vi "PicoScope6000Settings.vi"(4 "Channel D Settings":T2 {"Bandwidth" items=["Full", "20 MHz"]; "Range" items=["10 mV", "20 mV", "50 mV", "100 mV", "200 mV", "500 mV", "1 V", "2 V", "5 V", "10 V", "20 V", "50 V ", "100 V"]; "Coupling" items=["AC", "DC 1 MOhm", "DC 50 Ohm"]}, 5 "Channel B Settings":T2 {"Bandwidth" items=["Full", "20 MHz"]; "Range" items=["10 mV", "20 mV", "50 mV", "100 mV", "200 mV", "500 mV", "1 V", "2 V", "5 V", "10 V", "20 V", "50 V ", "100 V"]; "Coupling" items=["AC", "DC 1 MOhm", "DC 50 Ohm"]}, 6 "Channel C Settings":T2 {"Bandwidth" items=["Full", "20 MHz"]; "Range" items=["10 mV", "20 mV", "50 mV", "100 mV", "200 mV", "500 mV", "1 V", "2 V", "5 V", "10 V", "20 V", "50 V ", "100 V"]; "Coupling" items=["AC", "DC 1 MOhm", "DC 50 Ohm"]}, 7 "Channel A Settings":T2 {"Bandwidth" items=["Full", "20 MHz"]; "Range" items=["10 mV", "20 mV", "50 mV", "100 mV", "200 mV", "500 mV", "1 V", "2 V", "5 V", "10 V", "20 V", "50 V ", "100 V"]; "Coupling" items=["AC", "DC 1 MOhm", "DC 50 Ohm"]}, 8 "error in":errorcluster, 9 "Device Info":T1, 10 "Trigger Settings":T3 {"Trigger Direction" items=["Rising", "Falling"]}, 11 "handle in":i16) -> (0 "error out":errorcluster, 1 "Enabled array":i16[](array[numeric]), 3 "handle out":i16)   [LabVIEW 2009]
doc: "This VI is used to set up the oscilloscope. The inputs are clusters for setting channel and simple trigger settings. Advanced triggers can be set up using PicoScope6000AdvancedTriggerSettings.vi"
uses:
  ps6000.dll
  PicoScope6000AnalogChannelSettings.ctl
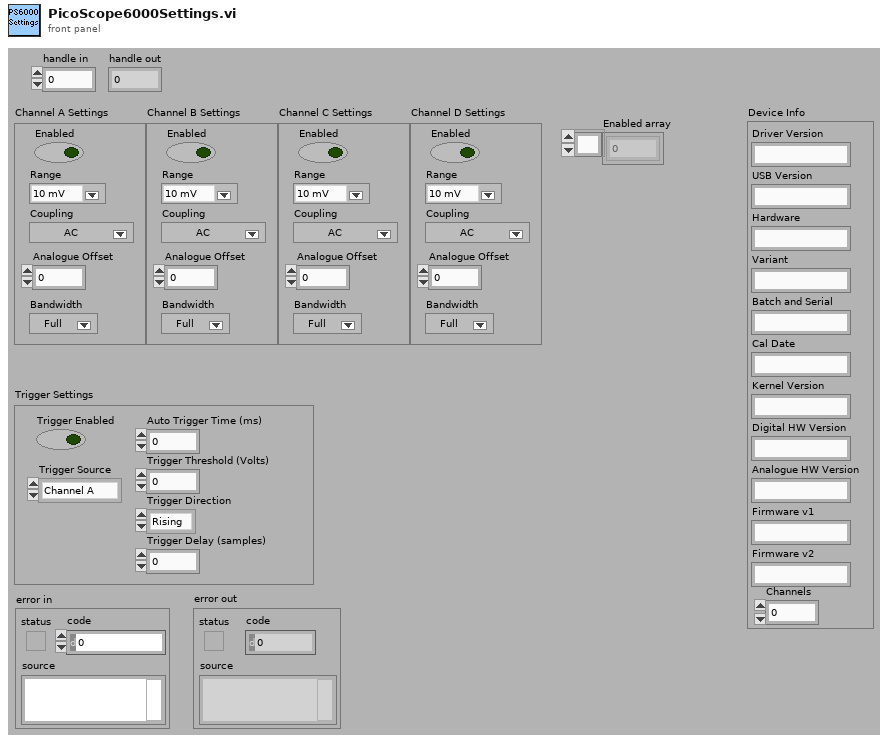
[diagram p1: front panel]
types:
  T1 = cluster{"Driver Version":string, "USB Version":string, "Hardware":string, "Variant":string, "Batch and Serial":string, "Cal Date":string, "Kernel Version":string, "Digital HW Version":string, "Analogue HW Version":string, "Firmware v1":string, "Firmware v2":string, "Channels":i16}
  T2 = typedef "PicoScope6000AnalogChannelSettings.ctl" = cluster{"Enabled":bool, "Coupling":u32, "Range":u32, "Analogue Offset":sgl, "Bandwidth":u32}
  T3 = cluster{"Trigger Enabled":bool, "Trigger Source":enum32{"Channel A", "Channel B", "Channel C", "Channel D", "External", "Aux."}, "Trigger Threshold (Volts)":dbl, "Trigger Direction":u16, "Trigger Delay (samples)":u32, "Auto Trigger Time (ms)":i16}
  T4 = cluster{"Enabled":bool, "Coupling":i32, "Range":u16, "Analogue Offset":sgl, "Bandwidth":i32}
  T5 = cluster{"Enabled":bool, "Coupling":u32, "Range":u32, "Analogue Offset":sgl, "Bandwidth":u32}
  T6 = cluster{"status":bool, "code":u32, "source":string}
  T7 = enum32{"Channel A", "Channel B", "Channel C", "Channel D", "External", "Aux."}
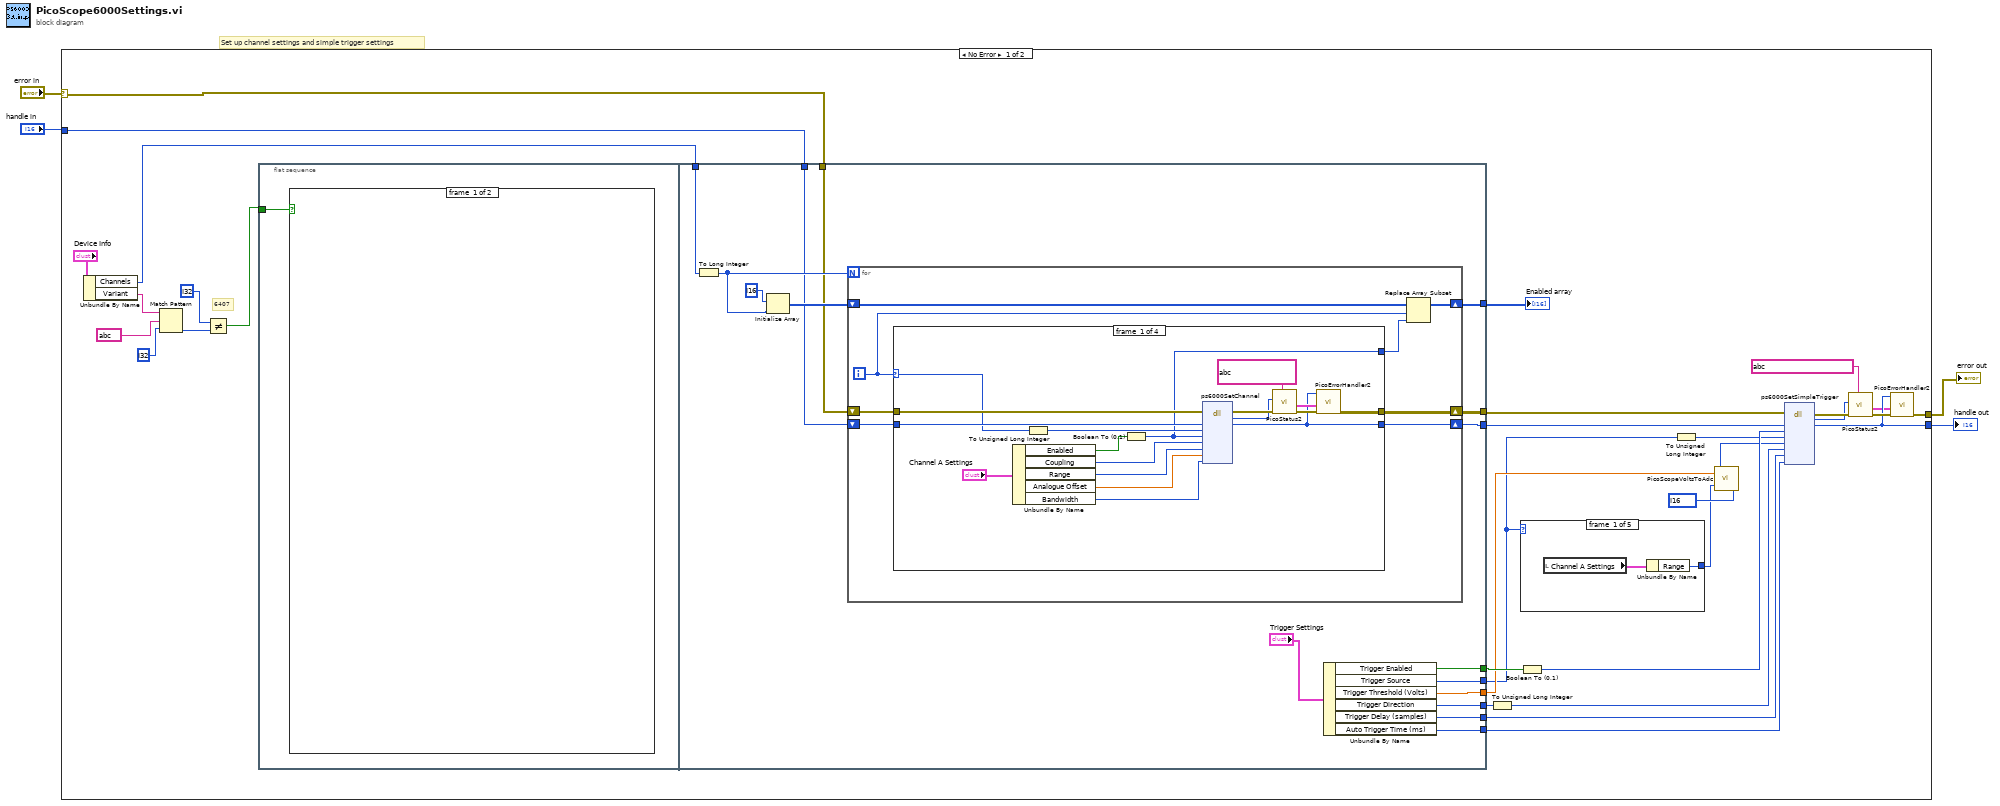
[diagram p0: block diagram]
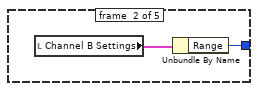
[diagram p2: hidden frame]
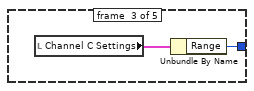
[diagram p3: hidden frame]
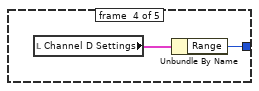
[diagram p4: hidden frame]
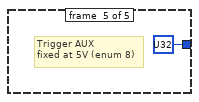
[diagram p5: hidden frame]
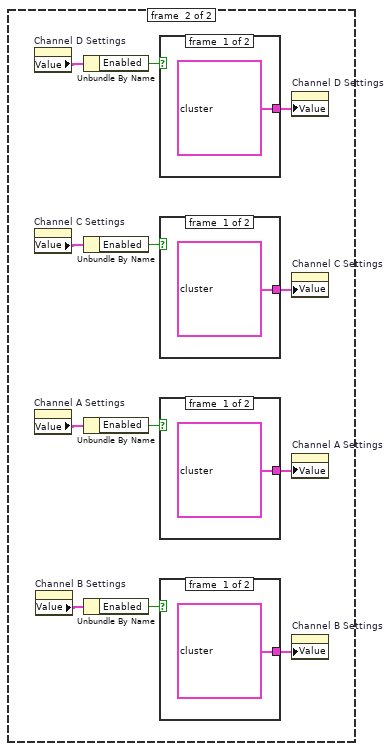
[diagram p6: hidden frame]
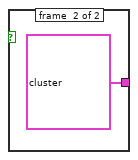
[diagram p7: hidden frame]
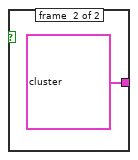
[diagram p8: hidden frame]
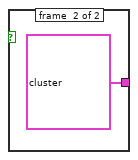
[diagram p9: hidden frame]
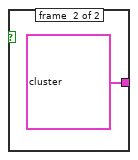
[diagram p10: hidden frame]
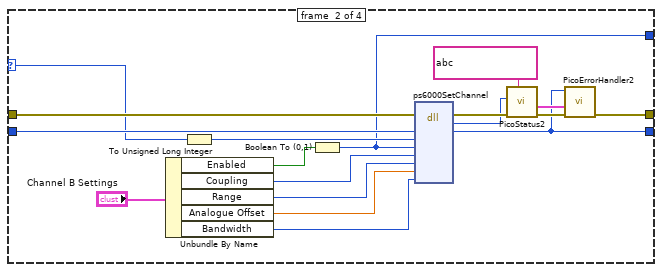
[diagram p11: hidden frame]
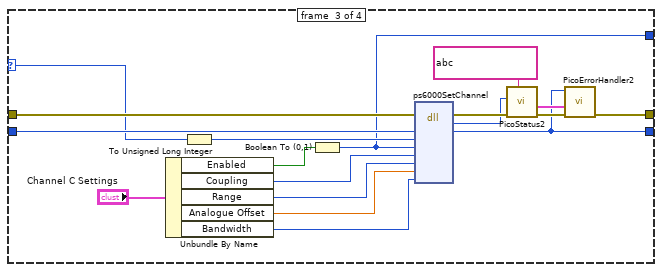
[diagram p12: hidden frame]
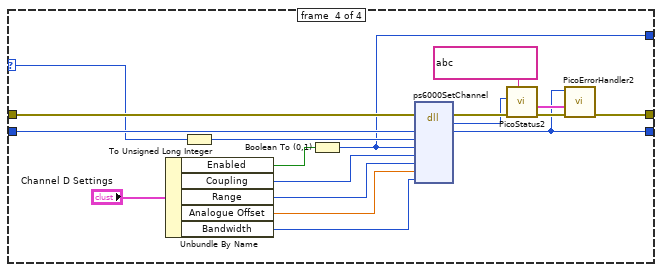
[diagram p13: hidden frame]
diagram:
  # "Set up channel settings and simple trigger settings"
  n1 = case shown="No Error" "error in" {
    selector: "error in" -> [w25 w164]
    tunnel: "handle in" -> [w24 w163]
    tunnel: [w31 w163] -> w2
    tunnel: [w32 w164] -> w1
    frame #0 {
      # "6407"
      n2 = Unbundle By Name("Device Info") -> ("Channels"=w6:i16, "Variant"=w12:string)
      n3 = Match Pattern(string=w12, regular expression=string ?, offset (0)=i32 ?) -> (offset past match=w11:i32)  [unwired: 3 out]
      n4 = Not Equal?(x=i32 ?, y=w11) -> (x != y?=w5:bool)
      n5 = flat-sequence {
        tunnel: w5 -> [w46]
        tunnel: [w79] -> w27
        tunnel: [w78] -> w26
        tunnel: [w77] -> w23
        tunnel: w25 -> [w76]
        tunnel: w24 -> [w75]
        tunnel: [w73] -> w20
        tunnel: [w72] -> w13
        tunnel: [w71] -> w19
        tunnel: [w70] -> w18
        tunnel: [w69] -> w17
        tunnel: [w68] -> w16
        tunnel: w6 -> [w67]
        frame #0 {
          n6 = case shown="True" w46 {
            frame #0 {
            }
            frame #1 {
              n7 = property on="Channel D Settings" class="Clust (strict)"() -> ("Value"=w48:T5)  [unwired: 2 in, 2 out]
              n8 = property on="Channel C Settings" class="Clust (strict)"() -> ("Value"=w50:T5)  [unwired: 2 in, 2 out]
              n9 = property on="Channel A Settings" class="Clust (strict)"() -> ("Value"=w55:T5)  [unwired: 2 in, 2 out]
              n10 = property on="Channel B Settings" class="Clust (strict)"() -> ("Value"=w53:T5)  [unwired: 2 in, 2 out]
              n11 = Unbundle By Name(w48) -> ("Enabled"=w57:bool)
              n12 = Unbundle By Name(w50) -> ("Enabled"=w58:bool)
              n13 = Unbundle By Name(w55) -> ("Enabled"=w56:bool)
              n14 = Unbundle By Name(w53) -> ("Enabled"=w52:bool)
              n15 = case shown="True" w57 {
                tunnel: [T4 ? ("Channel A Settings") T4 ? ("Channel A Settings")] -> w47
                frame #0 {
                }
                frame #1 {
                }
              }
              n16 = case shown="True" w58 {
                tunnel: [T4 ? ("Channel A Settings") T4 ? ("Channel A Settings")] -> w49
                frame #0 {
                }
                frame #1 {
                }
              }
              n17 = case shown="True" w56 {
                tunnel: [T4 ? ("Channel A Settings") T4 ? ("Channel A Settings")] -> w54
                frame #0 {
                }
                frame #1 {
                }
              }
              n18 = case shown="True" w52 {
                tunnel: [T4 ? ("Channel A Settings") T4 ? ("Channel A Settings")] -> w51
                frame #0 {
                }
                frame #1 {
                }
              }
              n19 = property on="Channel D Settings" class="Clust (strict)"("Value"=w47) -> ()  [unwired: 2 in, 2 out]
              n20 = property on="Channel C Settings" class="Clust (strict)"("Value"=w49) -> ()  [unwired: 2 in, 2 out]
              n21 = property on="Channel A Settings" class="Clust (strict)"("Value"=w54) -> ()  [unwired: 2 in, 2 out]
              n22 = property on="Channel B Settings" class="Clust (strict)"("Value"=w51) -> ()  [unwired: 2 in, 2 out]
            }
          }
        }
        frame #1 {
          n23 = To Long Integer(number=w67) -> (32bit integer=w81:i32)
          n24 = Initialize Array(i16 ? ("element"), w81) -> (w82:i16[])
          n25 = for {
            N: w81 -> [_]
            shift-right: [w89] -> w79
            shift-left: w76 -> [w90]
            shift-right: [w87] -> w78
            shift-left: w75 -> [w88]
            shift-right: [w85] -> w77
            shift-left: w82 -> [w86]
            i -> [w84]
            n26 = case shown="3" w84 {
              selector: w84 -> [w99 w117 w135 w153]
              tunnel: w90 -> [w103 w121 w139 w157]
              tunnel: [w102 w120 w138 w156] -> w89
              tunnel: w88 -> [w101 w119 w137 w155]
              tunnel: [w93 w111 w129 w147] -> w87
              tunnel: [w92 w110 w128 w146] -> w83
              frame #0 {
                n27 = Unbundle By Name("Channel A Settings") -> ("Enabled"=w98:bool, "Coupling"=w97:u32, "Range"=w96:u32, "Analogue Offset"=w95:sgl, "Bandwidth"=w94:u32)
                n28 = To Unsigned Long Integer(number=w99) -> (unsigned 32bit integer=w100:u32)
                n29 = Boolean To (0,1)(Boolean=w98) -> (0, 1=w92:i16)
                n30 = dll-call lib="PS6000.dll" fn="ps6000SetChannel" ("ps3000.dll:_ps3000_open_unit@0")(error in=w103, "handle"=w101, "channel"=w100, "enabled"=w92, "type"=w97, "range"=w96, "analogueOffset"=w95, "bandwidth"=w94) -> (error out=w108:errorcluster, "PICO_STATUS"=w106:u32, "handle"=w93:i16)  [unwired: 8 in, 1 out]
                n31 = call "PicoStatus2.vi"("PICO source"=string ? ("source"), "Error in"=w108, "PICO STATUS"=w106) -> ("error out"=w107:errorcluster, "PICO_STATUS out"=w105:T6)  [unwired: 5 in]
                n32 = call "PicoErrorHandler2.vi"("error in (no error)"=w107, "PICO_STATUS in"=w105, "handle In"=w93) -> ("error out"=w102:errorcluster)  [unwired: 8 in]
              }
              frame #1 {
                n33 = Unbundle By Name("Channel B Settings") -> ("Enabled"=w116:bool, "Coupling"=w115:u32, "Range"=w114:u32, "Analogue Offset"=w113:sgl, "Bandwidth"=w112:u32)
                n34 = To Unsigned Long Integer(number=w117) -> (unsigned 32bit integer=w118:u32)
                n35 = Boolean To (0,1)(Boolean=w116) -> (0, 1=w110:i16)
                n36 = dll-call lib="PS6000.dll" fn="ps6000SetChannel" ("ps3000.dll:_ps3000_open_unit@0")(error in=w121, "handle"=w119, "channel"=w118, "enabled"=w110, "type"=w115, "range"=w114, "analogueOffset"=w113, "bandwidth"=w112) -> (error out=w126:errorcluster, "PICO_STATUS"=w124:u32, "handle"=w111:i16)  [unwired: 8 in, 1 out]
                n37 = call "PicoStatus2.vi"("PICO source"=string ? ("source"), "Error in"=w126, "PICO STATUS"=w124) -> ("error out"=w125:errorcluster, "PICO_STATUS out"=w123:T6)  [unwired: 5 in]
                n38 = call "PicoErrorHandler2.vi"("error in (no error)"=w125, "PICO_STATUS in"=w123, "handle In"=w111) -> ("error out"=w120:errorcluster)  [unwired: 8 in]
              }
              frame #2 {
                n39 = Unbundle By Name("Channel C Settings") -> ("Enabled"=w134:bool, "Coupling"=w133:u32, "Range"=w132:u32, "Analogue Offset"=w131:sgl, "Bandwidth"=w130:u32)
                n40 = To Unsigned Long Integer(number=w135) -> (unsigned 32bit integer=w136:u32)
                n41 = Boolean To (0,1)(Boolean=w134) -> (0, 1=w128:i16)
                n42 = dll-call lib="PS6000.dll" fn="ps6000SetChannel" ("ps3000.dll:_ps3000_open_unit@0")(error in=w139, "handle"=w137, "channel"=w136, "enabled"=w128, "type"=w133, "range"=w132, "analogueOffset"=w131, "bandwidth"=w130) -> (error out=w144:errorcluster, "PICO_STATUS"=w142:u32, "handle"=w129:i16)  [unwired: 8 in, 1 out]
                n43 = call "PicoStatus2.vi"("PICO source"=string ? ("source"), "Error in"=w144, "PICO STATUS"=w142) -> ("error out"=w143:errorcluster, "PICO_STATUS out"=w141:T6)  [unwired: 5 in]
                n44 = call "PicoErrorHandler2.vi"("error in (no error)"=w143, "PICO_STATUS in"=w141, "handle In"=w129) -> ("error out"=w138:errorcluster)  [unwired: 8 in]
              }
              frame #3 {
                n45 = Unbundle By Name("Channel D Settings") -> ("Enabled"=w152:bool, "Coupling"=w151:u32, "Range"=w150:u32, "Analogue Offset"=w149:sgl, "Bandwidth"=w148:u32)
                n46 = To Unsigned Long Integer(number=w153) -> (unsigned 32bit integer=w154:u32)
                n47 = Boolean To (0,1)(Boolean=w152) -> (0, 1=w146:i16)
                n48 = dll-call lib="PS6000.dll" fn="ps6000SetChannel" ("ps3000.dll:_ps3000_open_unit@0")(error in=w157, "handle"=w155, "channel"=w154, "enabled"=w146, "type"=w151, "range"=w150, "analogueOffset"=w149, "bandwidth"=w148) -> (error out=w162:errorcluster, "PICO_STATUS"=w160:u32, "handle"=w147:i16)  [unwired: 8 in, 1 out]
                n49 = call "PicoStatus2.vi"("PICO source"=string ? ("source"), "Error in"=w162, "PICO STATUS"=w160) -> ("error out"=w161:errorcluster, "PICO_STATUS out"=w159:T6)  [unwired: 5 in]
                n50 = call "PicoErrorHandler2.vi"("error in (no error)"=w161, "PICO_STATUS in"=w159, "handle In"=w147) -> ("error out"=w156:errorcluster)  [unwired: 8 in]
              }
            }
            n51 = Replace Array Subset(array=w86, new element=w83, index=w84) -> (w85:i16[])
          }
          n52 = Unbundle By Name("Trigger Settings") -> ("Trigger Enabled"=w73:bool, "Trigger Source"=w72:T7, "Trigger Threshold (Volts)"=w71:dbl, "Trigger Direction"=w70:u16, "Trigger Delay (samples)"=w69:u32, "Auto Trigger Time (ms)"=w68:i16)
        }
      }
      n53 = To Unsigned Long Integer(number=w18) -> (unsigned 32bit integer=w36:u32)
      n54 = case shown="\"Channel D\"" w13 {
        tunnel: [w38 w40 w42 w44 u32 ? ("Range")] -> w15
        frame #0 {
          n55 = local read "Channel A Settings"() -> (w37:T2)
          n56 = Unbundle By Name(w37) -> ("Range"=w38:u32)
        }
        frame #1 {
          n57 = local read "Channel B Settings"() -> (w39:T2)
          n58 = Unbundle By Name(w39) -> ("Range"=w40:u32)
        }
        frame #2 {
          n59 = local read "Channel C Settings"() -> (w41:T2)
          n60 = Unbundle By Name(w41) -> ("Range"=w42:u32)
        }
        frame #3 {
          n61 = local read "Channel D Settings"() -> (w43:T2)
          n62 = Unbundle By Name(w43) -> ("Range"=w44:u32)
        }
        frame #4 {
          # "Trigger AUX\nfixed at 5V (enum 8)"
        }
      }
      n63 = Boolean To (0,1)(Boolean=w20) -> (0, 1=w35:i16)
      n64 = To Unsigned Long Integer(number=w13) -> (unsigned 32bit integer=w14:u32)
      n65 = call "PicoScopeVoltsToAdc.vi"("Max_adc"=i16 ? ("Max Adc value"), "Units"=w19, "Range Index"=w15) -> ("ADC count"=w22:i16)
      n66 = dll-call lib="PS6000.dll" fn="ps6000SetSimpleTrigger" ("ps3000.dll:_ps3000_open_unit@0")(error in=w27, "handle"=w26, "enabled"=w35, "source"=w14, "threshold"=w22, "direction"=w36, "delay"=w17, "autoTrigger_ms"=w16) -> (error out=w34:errorcluster, "PICO_STATUS"=w30:u32, "handle"=w31:i16)  [unwired: 8 in, 1 out]
      n67 = call "PicoStatus2.vi"("PICO source"=string ? ("source"), "Error in"=w34, "PICO STATUS"=w30) -> ("error out"=w33:errorcluster, "PICO_STATUS out"=w29:T6)  [unwired: 5 in]
      n68 = call "PicoErrorHandler2.vi"("error in (no error)"=w33, "PICO_STATUS in"=w29, "handle In"=w31) -> ("error out"=w32:errorcluster)  [unwired: 8 in]
      "Enabled array" <- w23
    }
    frame #1 {
    }
  }
  "handle out" <- w2
  "error out" <- w1
